vi "CONTROL_TRAYECTORIA.vi"() -> ()   [LabVIEW 2019]
uses:
  <vilib>/myRIO/Instrument Drivers/Onboard IO/PWM/typedefs/PWM Configuration.ctl
  <vilib>/myRIO/Instrument Drivers/Onboard IO/PWM/PWM.lvlib
  <vilib>/myRIO/Common/Instrument Driver Framework/myRIO v1.0/PWM/typedefs/PWM Channels Enum.ctl
  <vilib>/myRIO/Common/Instrument Driver Framework/Utilities/typedefs/Generic FPGA Reference.ctl
  <vilib>/myRIO/Common/Instrument Driver Framework/Utilities/typedefs/myRIO v1.0 Reference.ctl
  <vilib>/myRIO/Common/Instrument Driver Framework/Utilities/typedefs/Hardware Version Enum.ctl
  <vilib>/myRIO/Common/Instrument Driver Framework/Utilities/typedefs/myRIO Generic Hardware Reference.ctl
  <vilib>/myRIO/Instrument Drivers/Onboard IO/PWM/typedefs/PWM Reference.ctl
  <vilib>/myRIO/Instrument Drivers/Onboard IO/PWM/vis/Set Duty Cycle and Frequency.vi
  <vilib>/userDefined/High Color/nirio_resource_hc.ctl
  <vilib>/myRIO/Common/Instrument Driver Framework/myRIO v1.0/PWM/vis/myRIO v1.1 Open PWM.vi
  <vilib>/myRIO/Instrument Drivers/Onboard IO/PWM/vis/myRIO PWM Open.xnode
  <vilib>/myRIO/Common/Instrument Driver Framework/Utilities/vis/Is FPGA Ref Available.vi
  <vilib>/myRIO/Express VI/Onboard IO/PWM/PWM Express VI.xnode
  <vilib>/myRIO/Common/Instrument Driver Framework/myRIO v1.0/DIO/typedefs/DIO Channels Enum.ctl
  <vilib>/myRIO/Common/Instrument Driver Framework/myRIO v1.0/DIO/typedefs/DIO Channels List.ctl
  <vilib>/myRIO/Instrument Drivers/Onboard IO/DIO/typedefs/DIO Reference.ctl
  <vilib>/myRIO/Instrument Drivers/Onboard IO/DIO/DIO.lvlib
  <vilib>/myRIO/Instrument Drivers/Onboard IO/DIO/vis/Write.vi
  <vilib>/myRIO/Common/Instrument Driver Framework/myRIO v1.0/DIO/vis/myRIO v1.1 Open DIO.vi
  <vilib>/myRIO/Instrument Drivers/Onboard IO/DIO/vis/myRIO DIO Open.xnode
  <vilib>/myRIO/Express VI/Onboard IO/DO/DO Express VI.xnode
  <vilib>/myRIO/Instrument Drivers/Onboard IO/Encoder/Encoder.lvlib
  <vilib>/myRIO/Common/Instrument Driver Framework/myRIO v1.0/Encoder/typedefs/Encoder Channels Enum.ctl
  <vilib>/myRIO/Instrument Drivers/Onboard IO/Encoder/typedefs/Encoder Reference.ctl
  <vilib>/myRIO/Common/Instrument Driver Framework/myRIO v1.0/Encoder/typedefs/Encoder Signal Mode.ctl
  <vilib>/myRIO/Common/Instrument Driver Framework/myRIO v1.0/Encoder/typedefs/Encoder Configuration v1.0.ctl
  <vilib>/myRIO/Common/Instrument Driver Framework/myRIO v1.0/Encoder/vis/myRIO v1.1 Open Encoder.vi
  <vilib>/myRIO/Common/Instrument Driver Framework/myRIO v1.0/Encoder/vis/myRIO v1.0 Configure Encoder.vi
  <vilib>/myRIO/Instrument Drivers/Onboard IO/Encoder/vis/myRIO Encoder Open.xnode
panel:
  out "PWM_PI_Izq_Final_pct":dbl
  in  "Habilitar_PI_Izq":bool
  out "Bloquear_Integral_Izq":bool
  out "PI_Izq_Saturado":bool
  out "PWM_PI_Izq_Saturado_pct(x)":dbl
  in  "PWM_Limite_PI_Izq_pct":dbl
  out "Salida_PI_Izq":dbl
  out "Termino_I_Izq":dbl
  out "Incremento_Integral_Izq":dbl
  out "Termino_P_Izq":dbl
  in  "Ki_Vel_Izq":dbl
  in  "Kp_Vel_Izq":dbl
  out "Error_Velocidad_Der_m_s":dbl
  out "Error_Velocidad_Izq_m_s":dbl
  in  "Velocidad_Ref_Der_m_s":dbl
  in  "Velocidad_Ref_Izq_m_s":dbl
  out "Velocidad_Der_m_s":dbl
  out "Velocidad_Izq_m_s":dbl
  in  "stop":bool
  in  "Enum":T1(ring)
  in  "Duty Cycle (%)":dbl
  out "Encoder_Izq_Count":i32=30472
  out "Encoder_Der_Count":i32=-24622
  out "Delta_N_Izq":dbl
  out "Delta_N_Der":dbl
  out "Delta_t_ms":u32
  out "Delta_t_validado":dbl
  out "Tiempo_Valido":bool
  out "Delta_s_Izq_m":dbl
  out "Delta_s_Der_m":dbl
  out "Delta_s_Centro_m":dbl
  out "Delta_theta_rad":dbl
  out "Theta_Acumulado_rad":dbl
  out "Theta_Medio_rad":dbl
  out "Delta_X_m":dbl
  out "Delta_Y_m":dbl
  out "X_Actual_m":dbl
  out "Y_Actual_m":dbl
  out "Objetivo_25cm_Alcanzado":bool
  in  "Modo_Auto_25cm":bool
  out "Auto_Stop_25cm":bool
  out "Stop_25cm_Memorizado":bool
  in  "Distancia_Objetivo_m":dbl=0.25 format="%#_13g"
  in  "Modo_Auto_50cm":bool
  out "Objetivo_50cm_Alcanzado":bool
  out "Auto_Stop_50cm":bool
  out "Auto_Stop_General":bool
  out "Objetivo_360_Alcanzado":bool
  in  "Modo_Auto_Giro_360":bool
  out "Auto_Stop_Giro_360":bool
  out "Grafico_Posicion_X":dbl(graph)
  out "Grafico_Orientacion_rad":dbl(graph)
  out "Grafico_Trayectoria_XY":cluster{"X":dbl, "Y":dbl}[](graph)
  in  "RESET_GENERAL":bool
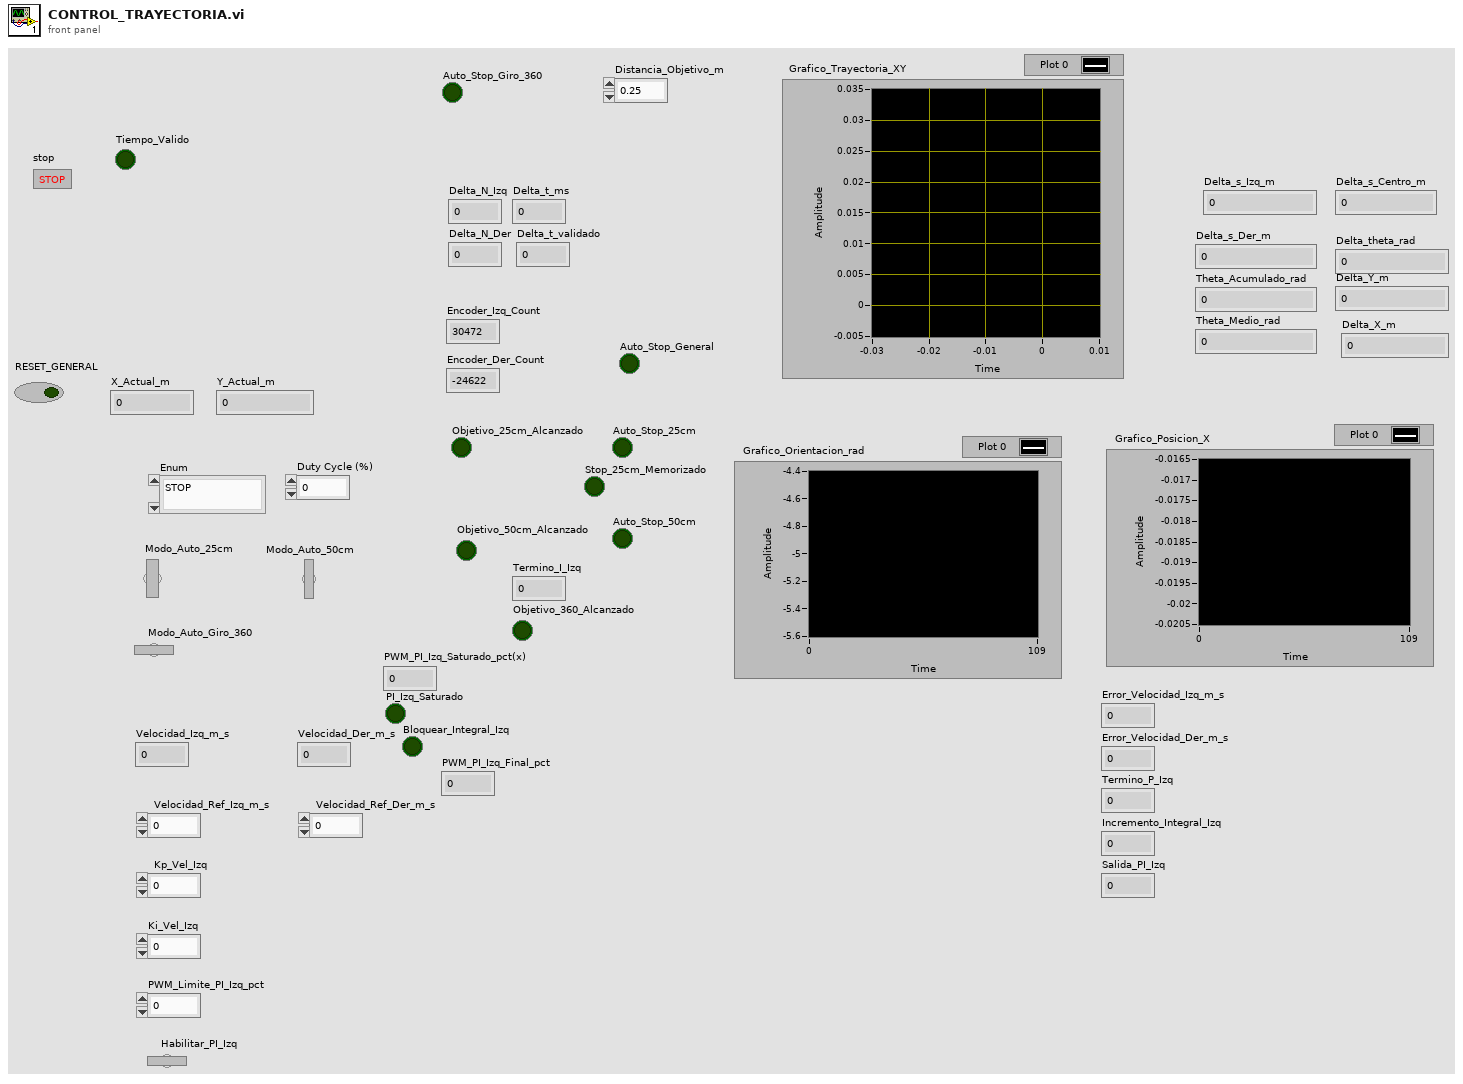
[diagram p1: front panel]
types:
  T1 = enum16{"STOP", "ADELANTE", "ATRÁS", "GIRO_IZQ", "GIRO_DER"}
  T2 = typedef "Encoder Signal Mode.ctl" = enum16{"Quadrature phase signal", "Step and direction signal"}
  T3 = typedef "Encoder.lvlib/Encoder Reference.ctl" = cluster{"myRIO Reference":T4, "Encoder Channels Enum":T8}
  T4 = typedef "myRIO Generic Hardware Reference.ctl" = cluster{"myRIO Model":T5, "myRIO Hardware Reference":T6}
  T5 = typedef "Hardware Version Enum.ctl" = enum16{"Unknown", "myRIO-1900", "myRIO-1950", "roboRIO", "NI ELVIS RIO CM", "ELVIS III"}
  T6 = typedef "myRIO v1.0 Reference.ctl" = cluster{"Generic FPGA Reference":T7, "Allow multiple opens":bool}
  T7 = typedef "Generic FPGA Reference.ctl" = refnum<k20>
  T8 = typedef "Encoder Channels Enum.ctl" = enum16{"Not Connected", "C/ENC0", "C/ENC1", "A/ENC", "A/ENC0", "A/ENC1", "A/ENC2", "A/ENC3", "A/ENC4", "A/ENC5", "A/ENC6", "A/ENC7", "A/ENC8", "A/ENC9", "B/ENC", "B/ENC0", "B/ENC1", "B/ENC2", "B/ENC3", "B/ENC4", "B/ENC5", "B/ENC6", "B/ENC7", "B/ENC8", "B/ENC9", "DIO/ENC0", "DIO/ENC1", "DIO/ENC2", "DIO/ENC3", "DIO/ENC4"}
  T9 = typedef "DIO.lvlib/DIO Reference.ctl" = cluster{"myRIO Reference":T4, "DIO Channels List":T10}
  T10 = typedef "DIO Channels List.ctl" = T11[]
  T11 = typedef "DIO Channels Enum.ctl" = enum16{"Not Connected", "C/DIO0", "C/DIO1", "C/DIO2", "C/DIO3", "C/DIO4", "C/DIO5", "C/DIO6", "C/DIO7", "A/DIO0", "A/DIO1", "A/DIO2", "A/DIO3", "A/DIO4", "A/DIO5", "A/DIO6", "A/DIO7", "A/DIO8", "A/DIO9", "A/DIO10", "A/DIO11", "A/DIO12", "A/DIO13", "A/DIO14", "A/DIO15", "A/DIO16", "A/DIO17", "A/DIO18", "A/DIO19", "B/DIO0", "B/DIO1", "B/DIO2", "B/DIO3", "B/DIO4", "B/DIO5", "B/DIO6", "B/DIO7", "B/DIO8", "B/DIO9", "B/DIO10", "B/DIO11", "B/DIO12", "B/DIO13", "B/DIO14", "B/DIO15", "B/DIO16", "B/DIO17", "B/DIO18", "B/DIO19", "LED0", "LED1", "LED2", "LED3", "Button0", "DIO/DIO0", "DIO/DIO1", "DIO/DIO2", "DIO/DIO3", "DIO/DIO4", "DIO/DIO5", "DIO/DIO6", "DIO/DIO7", "DIO/DIO8", "DIO/DIO9", "SPI/CS0", "SPI/CS1", "SPI/CS2", "SPI/CS3", "LED RADIO (Green)", "LED RADIO (Red)", "LED COMM (Green)", "LED COMM (Red)", "LED MODE (Green)", "LED MODE (Red)"}
  T12 = typedef "nirio_resource_hc.ctl" = tag
  T13 = typedef "PWM.lvlib/PWM Reference.ctl" = cluster{"myRIO Reference":T4, "PWM Channels Enum":T14, "PWM Configuration":T15}
  T14 = typedef "PWM Channels Enum.ctl" = enum16{"Not Connected", "C/PWM0", "C/PWM1", "A/PWM0", "A/PWM1", "A/PWM2", "A/PWM3", "A/PWM4", "A/PWM5", "A/PWM6", "A/PWM7", "A/PWM8", "A/PWM9", "A/PWM10", "A/PWM11", "A/PWM12", "A/PWM13", "A/PWM14", "A/PWM15", "A/PWM16", "A/PWM17", "A/PWM18", "A/PWM19", "B/PWM0", "B/PWM1", "B/PWM2", "B/PWM3", "B/PWM4", "B/PWM5", "B/PWM6", "B/PWM7", "B/PWM8", "B/PWM9", "B/PWM10", "B/PWM11", "B/PWM12", "B/PWM13", "B/PWM14", "B/PWM15", "B/PWM16", "B/PWM17", "B/PWM18", "B/PWM19", "PWM/PWM0", "PWM/PWM1", "PWM/PWM2", "PWM/PWM3", "PWM/PWM4", "PWM/PWM5", "PWM/PWM6", "PWM/PWM7", "PWM/PWM8", "PWM/PWM9"}
  T15 = typedef "PWM.lvlib/PWM Configuration.ctl" = cluster{"Frequency":dbl, "Duty Cycle":dbl}
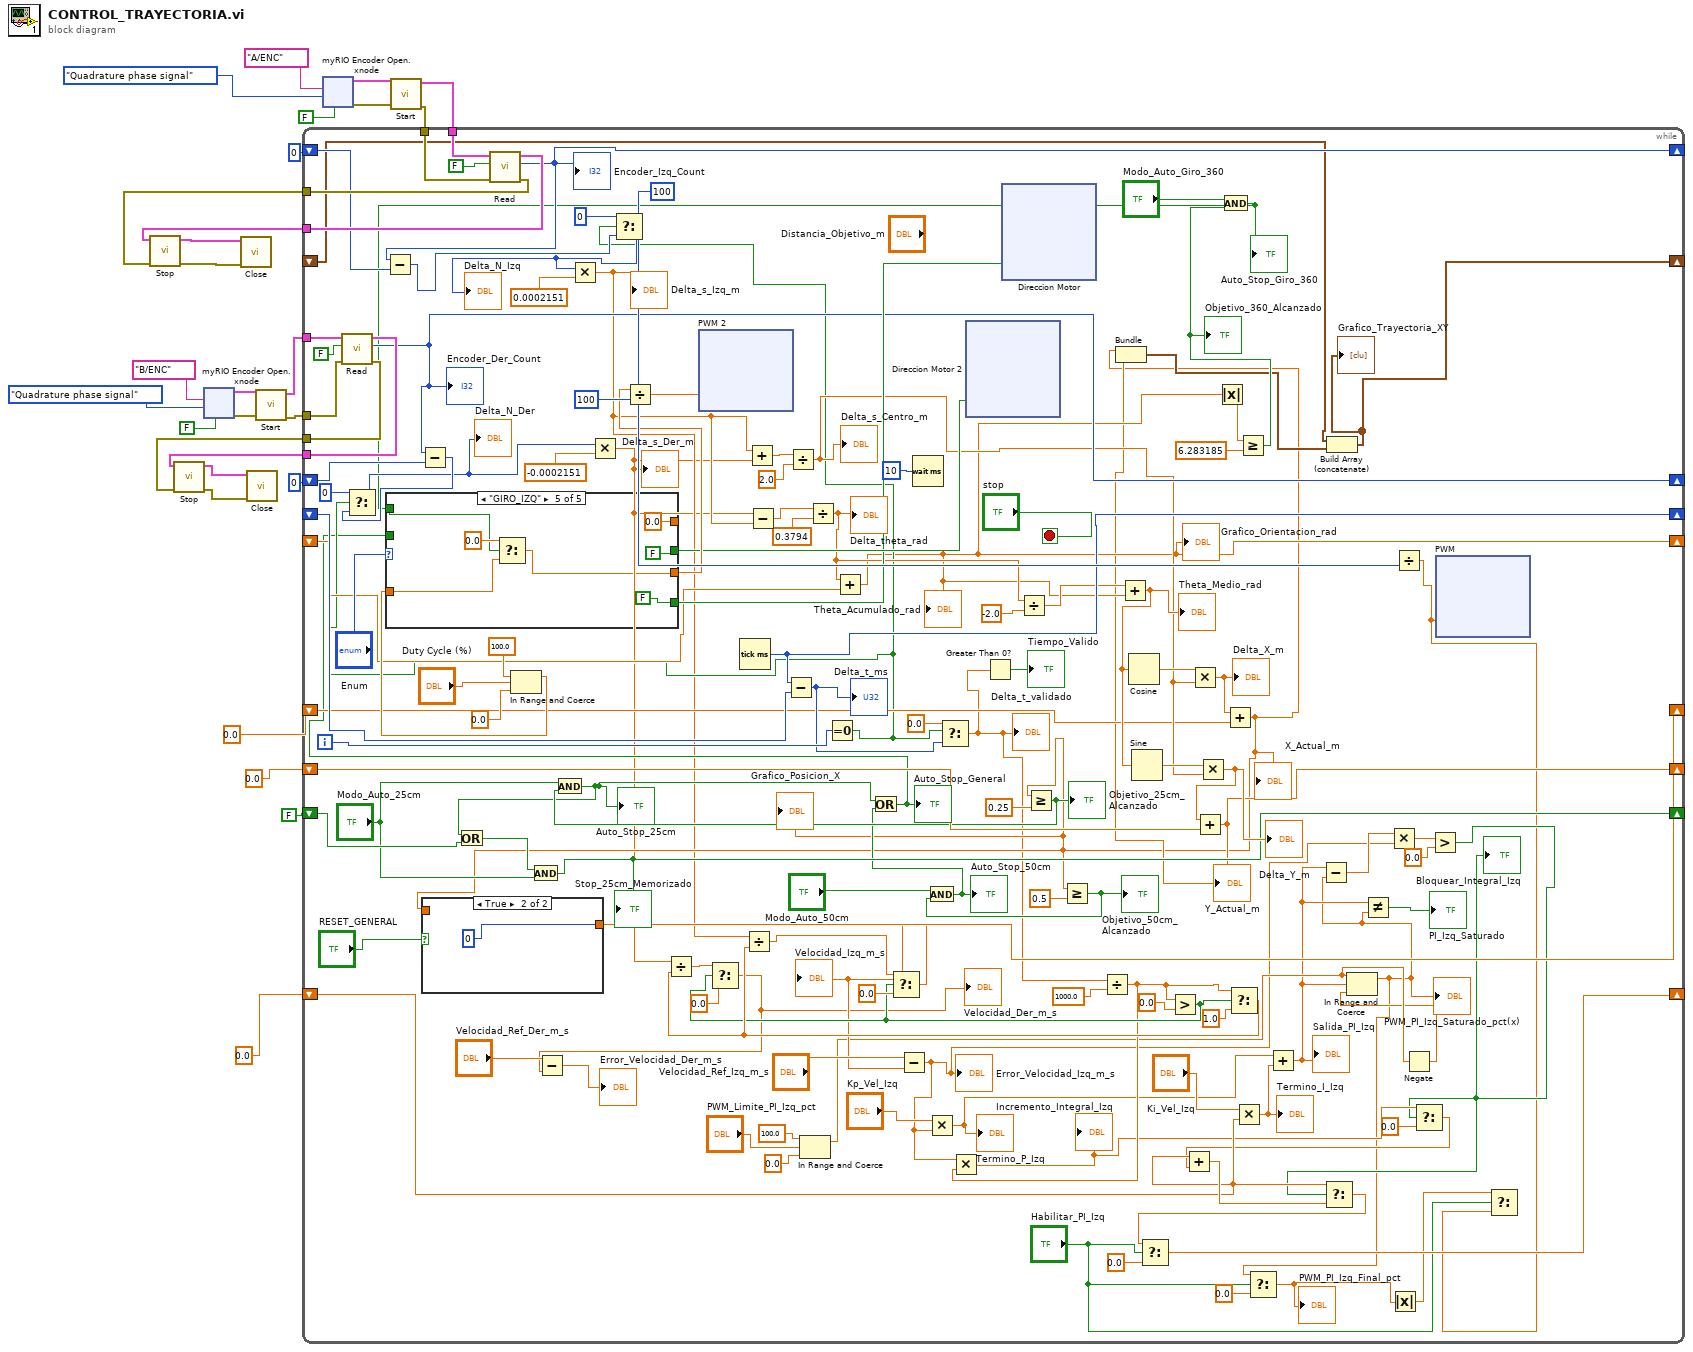
[diagram p0: block diagram]
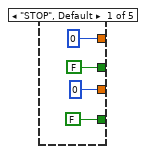
[diagram p3: hidden frame]
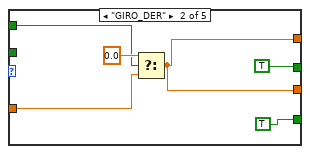
[diagram p4: hidden frame]
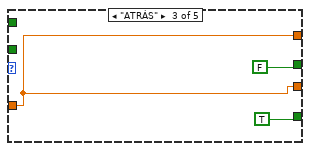
[diagram p5: hidden frame]
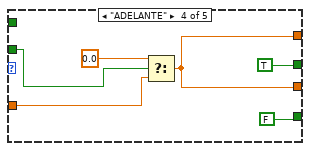
[diagram p6: hidden frame]
diagram:
  n1 = xnode "myRIO Encoder Open.xnode"("Channel Name"=tag "B/ENC", "Start Counter"=FALSE, "Encoder Signal Mode"=Encoder_Signal_Mode."Quadrature phase signal") -> ("error out"=w13:errorcluster, "Encoder Ref Out"=w14:T3)  [unwired: 2 in]
  n2 = call <vilib>:"Start.vi"("error in (no error)"=w13, "Encoder Ref In"=w14) -> ("error out"=w11:errorcluster, "Encoder Ref Out"=w12:T3)  [unwired: 8 in]
  n3 = xnode "myRIO Encoder Open.xnode"("Channel Name"=tag "A/ENC", "Start Counter"=FALSE, "Encoder Signal Mode"=Encoder_Signal_Mode."Quadrature phase signal") -> ("error out"=w24:errorcluster, "Encoder Ref Out"=w25:T3)  [unwired: 2 in]
  n4 = call <vilib>:"Start.vi"("error in (no error)"=w24, "Encoder Ref In"=w25) -> ("error out"=w22:errorcluster, "Encoder Ref Out"=w23:T3)  [unwired: 8 in]
  n5 = while {
    tunnel: w23 -> [w146]
    tunnel: w22 -> [w145]
    tunnel: [w143] -> w21
    tunnel: [w142] -> w20
    tunnel: w12 -> [w141]
    tunnel: w11 -> [w139]
    tunnel: [w138] -> w10
    tunnel: [w137] -> w9
    shift-right: [w136] -> _
    shift-left: 0 ("Counter Value") -> [w135]
    shift-right: [w133] -> _
    shift-left: 0 ("Counter Value") -> [w134]
    shift-right: [w132] -> _
    shift-left: _ -> [w131]
    shift-right: [w84] -> _
    shift-left: _ -> [w120]
    shift-right: [w78] -> _
    shift-left: 0.0 -> [w111]
    shift-right: [w83] -> _
    shift-left: 0.0 -> [w109]
    shift-right: [w97] -> _
    shift-left: FALSE -> [w100]
    shift-right: [w80] -> _
    shift-left: _ -> [w81]
    shift-right: [w35] -> _
    shift-left: 0.0 -> [w42]
    i -> [w129]
    stop <- "stop" stop-if-true
    n6 = call <vilib>:"Read.vi"("error in (no error)"=w139, "Reset Counter"=FALSE, "Encoder Ref In"=w141) -> ("error out"=w137:errorcluster, "Counter Value"=w133:i32, "Encoder Ref Out"=w138:T3)  [unwired: 4 in, 2 out]
    "Encoder_Der_Count" <- w133
    n7 = Subtract(x=w133, y=w134) -> (x-y=w103:i32)
    n8 = call <vilib>:"Read.vi"("error in (no error)"=w145, "Reset Counter"=FALSE, "Encoder Ref In"=w146) -> ("error out"=w142:errorcluster, "Counter Value"=w136:i32, "Encoder Ref Out"=w143:T3)  [unwired: 4 in, 2 out]
    "Encoder_Izq_Count" <- w136
    n9 = Subtract(x=w136, y=w135) -> (x-y=w107:i32)
    n10 = In Range and Coerce(upper limit=100.0, x="Duty Cycle (%)", lower limit=0.0) -> (coerced(x)=w147:dbl)  [unwired: 1 out]
    n11 = Tick Count (ms)() -> (millisecond timer value=w132:u32)
    n12 = Subtract(x=w132, y=w131) -> (x-y=w128:u32)
    "Delta_t_ms" <- w128
    n13 = In Range and Coerce(upper limit=100.0, x="PWM_Limite_PI_Izq_pct", lower limit=0.0) -> (coerced(x)=w51:dbl)  [unwired: 1 out]
    n14 = Equal To 0?(x=w129) -> (x = 0?=w104:bool)
    n15 = Select(t=0, s=w104, f=w103) -> (s? t:f=w102:i32)
    "Delta_N_Der" <- w102
    n16 = Multiply(x=w102, y=-0.0002151) -> (x*y=w69:dbl)
    "Delta_s_Der_m" <- w69
    n17 = Select(t=0, s=w104, f=w107) -> (s? t:f=w106:i32)
    "Delta_N_Izq" <- w106
    n18 = Multiply(x=w106, y=0.0002151) -> (x*y=w74:dbl)
    "Delta_s_Izq_m" <- w74
    n19 = Add(x=w74, y=w69) -> (x+y=w124:dbl)
    n20 = Subtract(x=w69, y=w74) -> (x-y=w122:dbl)
    n21 = Divide(x=w124, y=2.0) -> (x/y=w113:dbl)
    "Delta_s_Centro_m" <- w113
    n22 = Divide(x=w122, y=0.3794) -> (x/y=w119:dbl)
    "Delta_theta_rad" <- w119
    n23 = Add(x=w119, y=w120) -> (x+y=w84:dbl)
    "Theta_Acumulado_rad" <- w84
    "Grafico_Orientacion_rad" <- w84
    n24 = Wait (ms)(milliseconds to wait=10) -> ()  [unwired: 1 out]
    n25 = Select(t=0.0, s=w104, f=w128) -> (s? t:f=w76:dbl)
    "Delta_t_validado" <- w76
    n26 = Greater Than 0?(x=w76) -> (x > 0?=→"Tiempo_Valido":bool)
    n27 = Divide(x=w119, y=-2.0) -> (x/y=w117:dbl)
    n28 = Divide(x=w76, y=1000.0) -> (x/y=w58:dbl)
    n29 = Add(x=w117, y=w84) -> (x+y=w114:dbl)
    "Theta_Medio_rad" <- w114
    n30 = Cosine(x=w114) -> (cos(x)=w116:dbl)
    n31 = Sine(x=w114) -> (sin(x)=w115:dbl)
    n32 = Greater?(x=w58, y=0.0) -> (0:w65:bool)
    n33 = Multiply(x=w116, y=w113) -> (x*y=w112:dbl)
    "Delta_X_m" <- w112
    n34 = Multiply(x=w115, y=w113) -> (x*y=w110:dbl)
    "Delta_Y_m" <- w110
    n35 = Add(x=w110, y=w109) -> (x+y=w83:dbl)
    "Y_Actual_m" <- w83
    n36 = Absolute Value(x=w84) -> (abs(x)=w89:dbl)
    n37 = Add(x=w112, y=w111) -> (x+y=w77:dbl)
    "X_Actual_m" <- w77
    "Grafico_Posicion_X" <- w77
    n38 = case shown="True" "RESET_GENERAL" {
      tunnel: w77 -> [w160 _]
      tunnel: [w160 0] -> w78
      frame False {
      }
      frame True {
      }
    }
    n39 = Greater Or Equal?(x=w77, y=0.25) -> (x >= y?=w101:bool)
    "Objetivo_25cm_Alcanzado" <- w101
    n40 = And(x="Modo_Auto_25cm", y=w101) -> (x .and. y?=w91:bool)
    "Auto_Stop_25cm" <- w91
    n41 = Or(x=w91, y=w100) -> (x .or. y?=w98:bool)
    n42 = And(x=w98, y="Modo_Auto_25cm") -> (x .and. y?=w97:bool)
    "Stop_25cm_Memorizado" <- w97
    n43 = Greater Or Equal?(x=w77, y=0.5) -> (x >= y?=w94:bool)
    "Objetivo_50cm_Alcanzado" <- w94
    n44 = And(x="Modo_Auto_50cm", y=w94) -> (x .and. y?=w93:bool)
    "Auto_Stop_50cm" <- w93
    n45 = Or(x=w91, y=w93) -> (x .or. y?=w90:bool)
    "Auto_Stop_General" <- w90
    n46 = Bundle(w77, w83) -> (w82:cluster{dbl, dbl})  [unwired: 1 in]
    n47 = Select(t=w58, s=w65, f=1.0) -> (s? t:f=w68:dbl)
    n48 = Divide(x=w69, y=w68) -> (x/y=w67:dbl)
    n49 = Select(t=w67, s=w65, f=0.0) -> (s? t:f=w61:dbl)
    "Velocidad_Der_m_s" <- w61
    n50 = Subtract(x="Velocidad_Ref_Der_m_s", y=w61) -> (x-y=→"Error_Velocidad_Der_m_s":dbl)
    n51 = Divide(x=w74, y=w68) -> (x/y=w71:dbl)
    n52 = Select(t=w71, s=w65, f=0.0) -> (s? t:f=w63:dbl)
    "Velocidad_Izq_m_s" <- w63
    n53 = Subtract(x="Velocidad_Ref_Izq_m_s", y=w63) -> (x-y=w46:dbl)
    "Error_Velocidad_Izq_m_s" <- w46
    n54 = Multiply(x="Kp_Vel_Izq", y=w46) -> (x*y=w56:dbl)
    "Termino_P_Izq" <- w56
    n55 = Multiply(x=w46, y=w58) -> (x*y=w41:dbl)
    "Incremento_Integral_Izq" <- w41
    n56 = Multiply(x="Ki_Vel_Izq", y=w42) -> (x*y=w55:dbl)
    "Termino_I_Izq" <- w55
    n57 = Greater Or Equal?(x=w89, y=6.283185) -> (x >= y?=w86:bool)
    "Objetivo_360_Alcanzado" <- w86
    n58 = And(x="Modo_Auto_Giro_360", y=w86) -> (x .and. y?=w85:bool)
    "Auto_Stop_Giro_360" <- w85
    n59 = case shown="\"GIRO_IZQ\"" "Enum" {
      tunnel: [FALSE TRUE FALSE TRUE FALSE] -> w152
      tunnel: [0 w166 w172 w175 0.0 ("upper limit")] -> _
      tunnel: [0 w166 w172 w175 w182] -> w153
      tunnel: [FALSE TRUE TRUE FALSE FALSE] -> w151
      tunnel: w147 -> [_ w167 w172 w176 w183]
      tunnel: w90 -> [_ _ _ w177 _]
      tunnel: w85 -> [_ w168 _ _ w184]
      frame "STOP", Default {
      }
      frame "GIRO_DER" {
        n60 = Select(t=0.0, s=w168, f=w167) -> (s? t:f=w166:dbl)
      }
      frame "ATRÁS" {
      }
      frame "ADELANTE" {
        n61 = Select(t=0.0, s=w177, f=w176) -> (s? t:f=w175:dbl)
      }
      frame "GIRO_IZQ" {
        n62 = Select(t=0.0, s=w184, f=w183) -> (s? t:f=w182:dbl)
      }
    }
    n63 = Divide(x=w153, y=100) -> (x/y=w157:dbl)
    n64 = xnode "PWM 2"("Duty Cycle"=w157) -> ()  [unwired: 1 in, 1 out]
    n65 = xnode "Direccion Motor 2"("A/DIO0 (Pin 11)"=w152) -> ()  [unwired: 1 in, 1 out]
    n66 = xnode "Direccion Motor"("B/DIO0 (Pin 11)"=w151) -> ()  [unwired: 1 in, 1 out]
    n67 = Add(x=w56, y=w55) -> (x+y=w48:dbl)
    "Salida_PI_Izq" <- w48
    n68 = Build Array (concatenate)(w81, w82) -> (w80:cluster{dbl, dbl}[])
    "Grafico_Trayectoria_XY" <- w80
    n69 = Divide(y=100) -> (x/y=w29:dbl)  [unwired: 1 in]
    n70 = Negate(x=w51) -> (-x=w50:dbl)
    n71 = In Range and Coerce(upper limit=w51, x=w48, lower limit=w50) -> (coerced(x)=w34:dbl)  [unwired: 1 out]
    "PWM_PI_Izq_Saturado_pct(x)" <- w34
    n72 = Select(t=w34, s="Habilitar_PI_Izq", f=0.0) -> (s? t:f=w32:dbl)
    "PWM_PI_Izq_Final_pct" <- w32
    n73 = Subtract(x=w48, y=w34) -> (x-y=w47:dbl)
    n74 = Not Equal?(x=w48, y=w34) -> (x != y?=→"PI_Izq_Saturado":bool)
    n75 = Multiply(x=w47, y=w46) -> (x*y=w45:dbl)
    n76 = Absolute Value(x=w32) -> (abs(x)=w31:dbl)
    n77 = Greater?(x=w45, y=0.0) -> (0:w39:bool)
    "Bloquear_Integral_Izq" <- w39
    n78 = Select(t=w41, s=w39, f=0.0) -> (s? t:f=w38:dbl)
    n79 = Add(x=w42, y=w38) -> (x+y=w43:dbl)
    n80 = Select(t=w42, s=w39, f=w43) -> (s? t:f=w37:dbl)
    n81 = Select(t=w37, s="Habilitar_PI_Izq", f=0.0) -> (s? t:f=w35:dbl)
    n82 = xnode "PWM"("Duty Cycle"=w29) -> ()  [unwired: 1 in, 1 out]
    n83 = Select(t=w31, s="Habilitar_PI_Izq", f=w29) -> ()  [unwired: 1 out]
  }
  n84 = call <vilib>:"Stop.vi"("error in (no error)"=w20, "Encoder Ref In"=w21) -> ("error out"=w18:errorcluster, "Encoder Ref Out"=w19:T3)  [unwired: 8 in]
  n85 = call <vilib>:"Stop.vi"("error in (no error)"=w9, "Encoder Ref In"=w10) -> ("error out"=w7:errorcluster, "Encoder Ref Out"=w8:T3)  [unwired: 8 in]
  n86 = call <vilib>:"Close.vi"("error in (no error)"=w18, "Encoder Ref In"=w19) -> ()  [unwired: 9 in, 1 out]
  n87 = call <vilib>:"Close.vi"("error in (no error)"=w7, "Encoder Ref In"=w8) -> ()  [unwired: 9 in, 1 out]
